vi "Toast With Link Button.vi"(8 "error in":errorcluster) -> (0 "error out":errorcluster, 3 "Toast XML":string)   [LabVIEW 2026]
doc: "Open a web page from a Windows toast button. Click Open project on GitHub to let Windows open the link in your browser. This button uses protocol activation. Press Stop in LabVIEW to close the example."
uses:
  ActivationHandler/ActivationHandler.lvclass
  ToastBuilder/ToastBuilder.lvclass
  ToastBuilder/Create ToastBuilder.vi
  ToastService/ToastService.lvclass
  ToastNotification/ToastNotification.lvlib
panel:
  in  "stop":bool
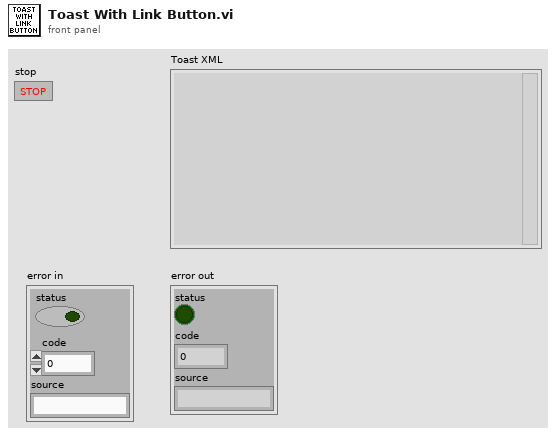
[diagram p1: front panel]
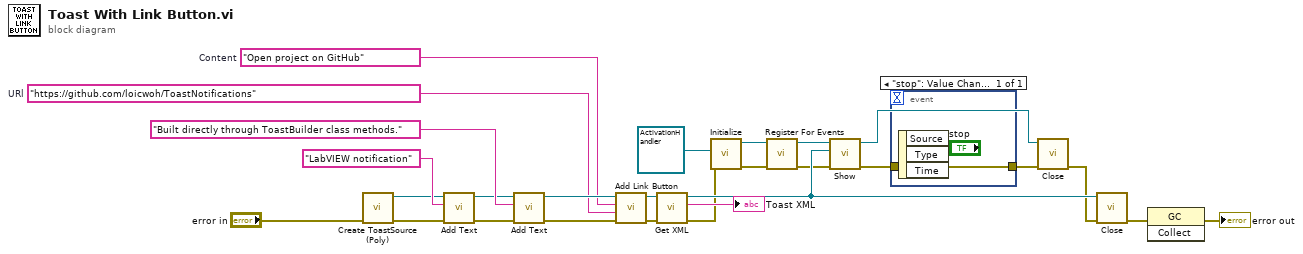
[diagram p0: block diagram]
diagram:
  w2 = "https://github.com/loicwoh/ToastNotifications"  # URl
  w3 = "Open project on GitHub"  # Content
  n1 = call-poly "Create ToastSource (Poly).vi"("error in"="error in") -> ("error out"=w22:errorcluster, "ToastBuilder out"=w21:refnum<class "ToastBuilder.lvclass">)  [unwired: 9 in]
  n2 = call "Add Text.vi"("error in"=w22, "text"="LabVIEW notification", "ToastBuilder in"=w21) -> ("error out"=w25:errorcluster, "ToastBuilder out"=w24:refnum<class "ToastBuilder.lvclass">)  [unwired: 7 in]
  n3 = call "Add Text.vi"("error in"=w25, "text"="Built directly through ToastBuilder class methods.", "ToastBuilder in"=w24) -> ("error out"=w6:errorcluster, "ToastBuilder out"=w7:refnum<class "ToastBuilder.lvclass">)  [unwired: 7 in]
  n4 = call "Add Link Button.vi"("error in (no error)"=w6, "URl"=w2, "Content"=w3, "ToastBuilder in"=w7) -> ("error out"=w5:errorcluster, "ToastBuilder out"=w4:refnum<class "ToastBuilder.lvclass">)  [unwired: 6 in]
  n5 = call-dynamic "Get XML.vi"("error in"=w5, "ToastBuilder in"=w4) -> ("error out"=w18:errorcluster, "GetContent"=→"Toast XML":string, "ToastBuilder out"=w19:refnum<class "ToastBuilder.lvclass">)  [unwired: 7 in]
  n6 = call "Initialize.vi"("error in (no error)"=w18, "ActivationHandler in"=refnum<class "ActivationHandler.lvclass"> refnum) -> ("error out"=w16:errorcluster, "ToastService out"=w14:refnum<class "ToastService.lvclass">)  [unwired: 7 in, 1 out]
  n7 = call "Register For Events.vi"("error in (no error)"=w16, "ToastService in"=w14) -> ("error out"=w15:errorcluster, "ToastService out"=w13:refnum<class "ToastService.lvclass">)  [unwired: 8 in]
  n8 = call "Show.vi"("error in (no error)"=w15, "ToastSource in"=w19, "ToastService in"=w13) -> ("error out"=w12:errorcluster, "ToastService out"=w10:refnum<class "ToastService.lvclass">)  [unwired: 7 in]
  n9 = event shown="[0] \"stop\": Value Change" {
    selector: _ -> [_]
    dyn-events: _ -> [_]
    timeout: _ -> [_]
    tunnel: [w28] -> w11
    tunnel: w12 -> [w28]
    event "stop": Value Change {
      n10 = event-data() -> ()  [unwired: 1 in, 3 out]
    }
  }
  n11 = call "Close.vi"("error in (no error)"=w11, "ToastService in"=w10) -> ("error out"=w17:errorcluster)  [unwired: 9 in]
  n12 = call-dynamic "Close.vi"("error in"=w17, "ToastBuilder in"=w19) -> ("error out"=w9:errorcluster)  [unwired: 9 in]
  n13 = invoke class="GC" method="Collect"(error in=w9) -> (error out=→"error out":errorcluster)  [unwired: 2 in, 2 out]
